vi "Find Item in Library.vi"(7 "Item Type":string, 8 "error in (no error)":errorcluster, 10 "Item Name":string, 11 "Library item in":refnum<vi>) -> (0 "error out":errorcluster, 1 "Found?":bool, 2 "Project Item (Library Item)":refnum<vi>, 3 "Library item out":refnum<vi>)   [LabVIEW 2019, in "gRPC Template Creation Utility.lvlib"]
uses:
  gRPC Template Creation Utility.lvlib
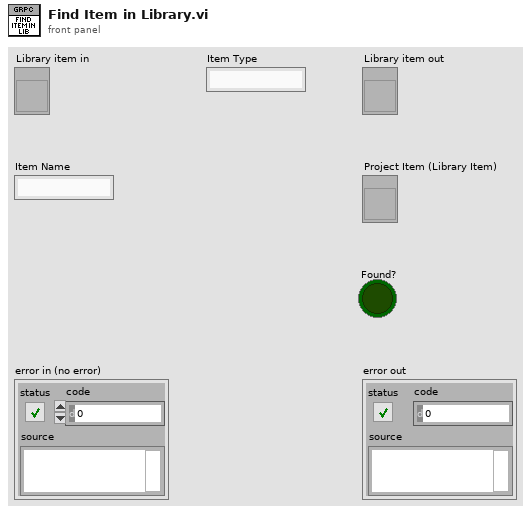
[diagram p1: front panel]
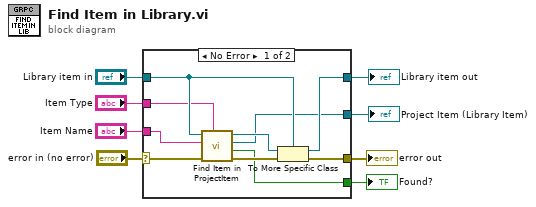
[diagram p0: block diagram]
diagram:
  n1 = case shown="No Error" "error in (no error)" {
    selector: "error in (no error)" -> [w9 w19]
    tunnel: "Item Name" -> [w10 _]
    tunnel: "Item Type" -> [w11 _]
    tunnel: "Library item in" -> [w16 w20]
    tunnel: [w17 w20] -> w2
    tunnel: [w12 _] -> w4
    tunnel: [w13 _] -> w3
    tunnel: [w14 w19] -> w1
    frame No Error {
      n2 = call "Find Item in ProjectItem.vi"("Item Type"=w11, "error in (no error)"=w9, "Name"=w10, "ProjectItem in"=w16) -> ("error out"=w15:errorcluster, "Found ?"=w12:bool, "Item Refnum out"=w13:refnum<vi>, "ProjectItem out"=w18:refnum<vi>)  [unwired: 4 in]
      n3 = To More Specific Class(target class=w16, reference=w18, error in=w15) -> (specific class reference=w17:refnum<vi>, error out=w14:errorcluster)
    }
    frame Error {
    }
  }
  "Project Item (Library Item)" <- w3
  "Found?" <- w4
  "Library item out" <- w2
  "error out" <- w1
